vi "RemoteVI Highlight Menu Row.vi"(0 "hWnd":u64, 5 "menu":u64, 7 "y":i32, 9 "probe?":bool=TRUE, 11 "error in":errorcluster) -> (4 "keyed?":bool, 6 "hit?":bool, 8 "top":i32, 10 "bottom":i32, 15 "error out":errorcluster)   [LabVIEW 2020, in "RemoteVI.lvlib"]
doc: "Moves the highlight of an open LabVIEW menu onto the item at window row y WITHOUT moving the host cursor or the menu: LabVIEW menus take VK_DOWN / VK_UP posted to the panel window (RemoteVI Post Menu Key.vi), so the menu is captured (RemoteVI Menu Highlight.vi), the highlighted band is compared with y and one key is posted towards it, until the band contains y (hit? TRUE). It stops without a hit when the band did not move after a key (nothing selectable further on), when it jumped past y (y lies on a separator or a disabled item), or after 100 keys. Menus wrap around at the ends (measured); a wrap is undone with one key in the other direction and ends the search. When nothing is highlighted yet, probe? is TRUE and the window has the menu background colour (RemoteVI Menu Highlight.vi menu colours? - a key posted into the colour picker spoils its next click, measured), one key is posted first (it is not a step: where it lands depends on the menu - a ring menu highlights its first item for VK_UP too, measured - so no wrap or overshoot is concluded from it) - VK_DOWN when y lies in the upper half (it highlights the first item), VK_UP otherwise (the last item); when that still shows no highlight the window is no keyboard menu (colour picker, line width popup) and keyed? is FALSE. top and bottom are the band last seen, in window pixels. After each key the menu is captured until its highlight moved (RemoteVI Wait Highlight Change.vi, at most 120 ms) - the repaint can lag the key by 100 ms (measured), and reading the old highlight would end the search one item short. Win32 only, no VI Server call, so it runs while the menu's modal loop holds LabVIEW's UI thread."
uses:
  RemoteVI.lvlib
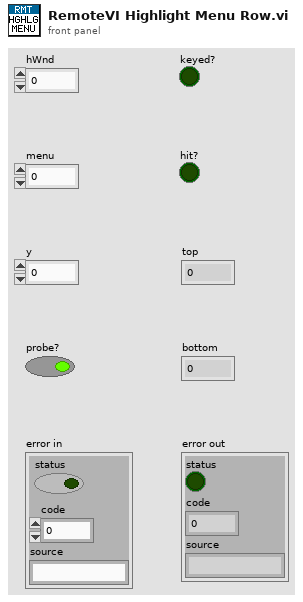
[diagram p1: front panel]
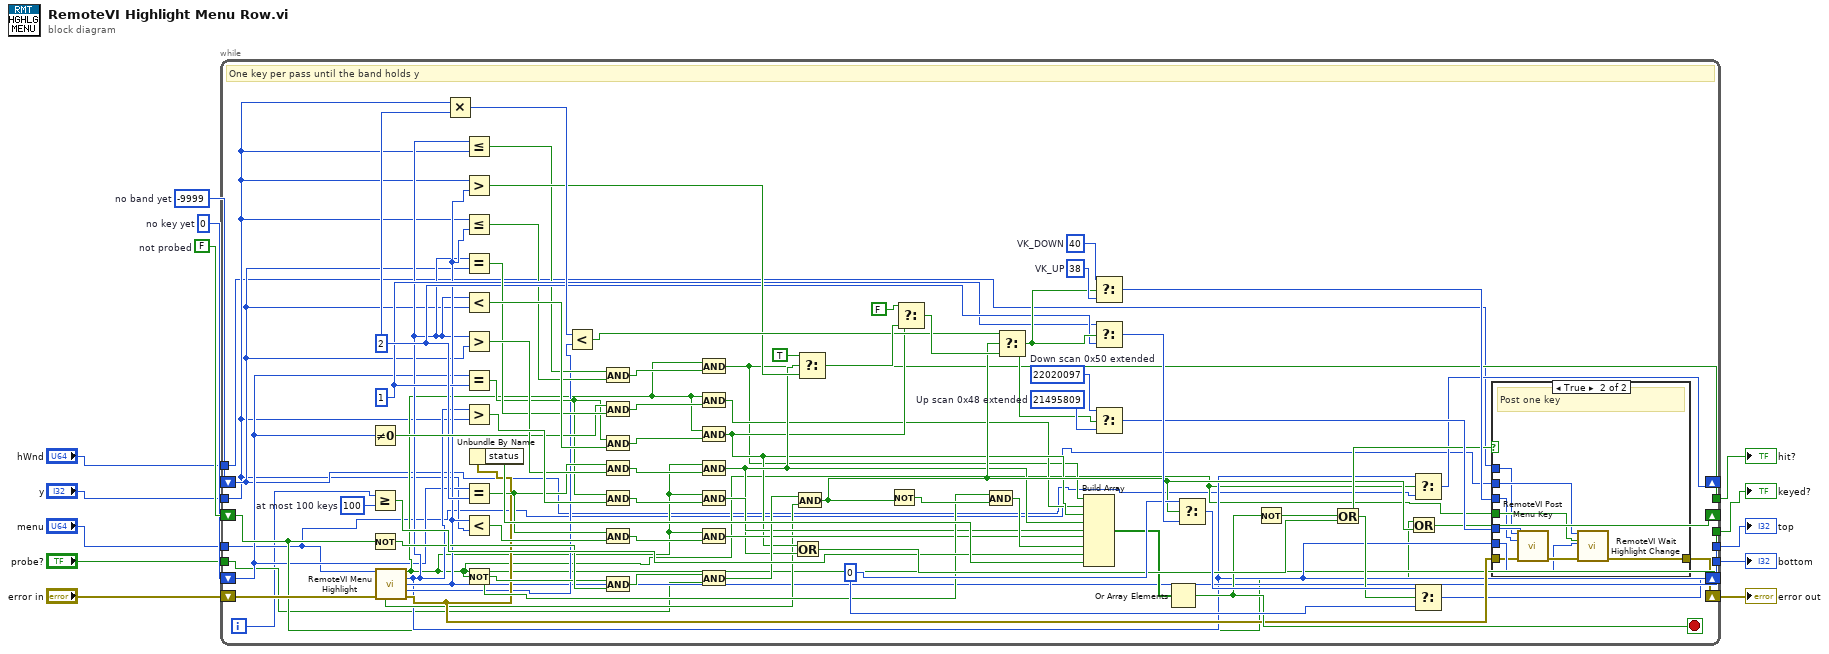
[diagram p0: block diagram]
diagram:
  w8 = FALSE  # not probed
  w7 = 0  # no key yet
  w6 = -9999  # no band yet
  n1 = while {
    tunnel: "hWnd" -> [w15]
    tunnel: "menu" -> [w16]
    tunnel: "y" -> [w17]
    tunnel: "probe?" -> [w18]
    shift-right: [w20] -> _
    shift-left: w6 -> [w19]
    shift-right: [w22] -> _
    shift-left: w7 -> [w21]
    shift-right: [w24] -> _
    shift-left: w8 -> [w23]
    shift-right: [w26] -> w9
    shift-left: "error in" -> [w25]
    tunnel: [w27] -> w10
    tunnel: [w28] -> w12
    tunnel: [w29] -> w13
    tunnel: [w36] -> w11
    i -> [w14]
    stop <- w68 stop-if-true
    w86 = 0
    w83 = i64 21495809  # Up scan 0x48 extended
    w82 = i64 22020097  # Down scan 0x50 extended
    w81 = u64 38  # VK_UP
    w80 = u64 40  # VK_DOWN
    w64 = 100  # at most 100 keys
    w38 = 2
    w37 = 1
    # "One key per pass until the band holds y"
    n2 = Not Equal To 0?(x=w21) -> (x != 0?=w41:bool)
    n3 = Greater Or Equal?(x=w14, y=w64) -> (x >= y?=w65:bool)
    n4 = Not(x=w23) -> (.not. x?=w58:bool)
    n5 = call "RemoteVI Menu Highlight.vi"("hwnd"=w16, "error in"=w25) -> ("found?"=w27:bool, "top"=w28:i32, "bottom"=w29:i32, "height"=w30:i32, "menu colours?"=w31:bool, "error out"=w32:errorcluster)  [unwired: 8 in]
    n6 = Multiply(x=w17, y=w38) -> (x*y=w70:i32)
    n7 = Less Or Equal?(x=w28, y=w17) -> (x <= y?=w33:bool)
    n8 = Greater?(x=w17, y=w29) -> (0:w69:bool)
    n9 = Less Or Equal?(x=w17, y=w29) -> (x <= y?=w34:bool)
    n10 = Equal?(x=w28, y=w19) -> (x = y?=w42:bool)
    n11 = Less?(x=w28, y=w19) -> (x < y?=w45:bool)
    n12 = Greater?(x=w28, y=w19) -> (0:w46:bool)
    n13 = Equal?(x=w21, y=w37) -> (x = y?=w39:bool)
    n14 = Greater?(x=w28, y=w17) -> (0:w51:bool)
    n15 = Equal?(x=w21, y=w38) -> (x = y?=w40:bool)
    n16 = Less?(x=w29, y=w17) -> (x < y?=w54:bool)
    n17 = Not(x=w27) -> (.not. x?=w57:bool)
    n18 = Unbundle By Name(w32) -> ("status"=w66:bool)
    n19 = Less?(x=w70, y=w30) -> (x < y?=w71:bool)
    n20 = And(x=w33, y=w34) -> (x .and. y?=w35:bool)
    n21 = And(x=w41, y=w42) -> (x .and. y?=w43:bool)
    n22 = And(x=w39, y=w45) -> (x .and. y?=w47:bool)
    n23 = And(x=w40, y=w46) -> (x .and. y?=w49:bool)
    n24 = And(x=w39, y=w51) -> (x .and. y?=w52:bool)
    n25 = And(x=w40, y=w54) -> (x .and. y?=w55:bool)
    n26 = And(x=w57, y=w58) -> (x .and. y?=w59:bool)
    n27 = And(x=w27, y=w35) -> (x .and. y?=w36:bool)
    n28 = And(x=w27, y=w43) -> (x .and. y?=w44:bool)
    n29 = And(x=w27, y=w47) -> (x .and. y?=w48:bool)
    n30 = And(x=w27, y=w49) -> (x .and. y?=w50:bool)
    n31 = And(x=w27, y=w52) -> (x .and. y?=w53:bool)
    n32 = And(x=w27, y=w55) -> (x .and. y?=w56:bool)
    n33 = And(x=w59, y=w18) -> (x .and. y?=w60:bool)
    n34 = Or(x=w48, y=w50) -> (x .or. y?=w78:bool)
    n35 = And(x=w60, y=w31) -> (x .and. y?=w61:bool)
    n36 = Select(t=TRUE, s=w50, f=w69) -> (s? t:f=w74:bool)
    n37 = Not(x=w61) -> (.not. x?=w62:bool)
    n38 = Select(t=FALSE, s=w48, f=w74) -> (s? t:f=w75:bool)
    n39 = And(x=w57, y=w62) -> (x .and. y?=w63:bool)
    n40 = Select(t=w71, s=w61, f=w75) -> (s? t:f=w76:bool)
    n41 = Build Array(w36, w44, w48, w50, w53, w56, w63, w65, w66) -> (w67:bool[])
    n42 = Select(t=w80, s=w76, f=w81) -> (s? t:f=w84:u64)
    n43 = Select(t=w37, s=w76, f=w38) -> (s? t:f=w87:i32)
    n44 = Select(t=w82, s=w76, f=w83) -> (s? t:f=w85:i64)
    n45 = Or Array Elements(Boolean array=w67) -> (logical OR=w68:bool)
    n46 = Select(t=w86, s=w61, f=w87) -> (s? t:f=w88:i32)
    n47 = Not(x=w68) -> (.not. x?=w77:bool)
    n48 = Or(x=w77, y=w78) -> (x .or. y?=w79:bool)
    n49 = Or(x=w23, y=w61) -> (x .or. y?=w24:bool)
    n50 = Select(t=w28, s=w27, f=w19) -> (s? t:f=w20:i32)
    n51 = Select(t=w88, s=w79, f=w86) -> (s? t:f=w22:i32)
    n52 = case shown="True" w79 {
      tunnel: w15 -> [_ w91]
      tunnel: w16 -> [_ w94]
      tunnel: w32 -> [w89 w90]
      tunnel: w27 -> [_ w95]
      tunnel: w28 -> [_ w96]
      tunnel: w84 -> [_ w92]
      tunnel: w85 -> [_ w93]
      tunnel: [w89 w98] -> w26
      frame False {
      }
      frame True {
        # "Post one key"
        n53 = call "RemoteVI Post Menu Key.vi"("hWnd"=w91, "vk"=w92, "key lParam"=w93, "error in"=w90) -> ("error out"=w97:errorcluster)  [unwired: 11 in]
        n54 = call "RemoteVI Wait Highlight Change.vi"("menu"=w94, "found before"=w95, "top before"=w96, "error in"=w97) -> ("error out"=w98:errorcluster)  [unwired: 10 in, 1 out]
      }
    }
  }
  "keyed?" <- w10
  "hit?" <- w11
  "top" <- w12
  "bottom" <- w13
  "error out" <- w9
